vi "PicoScope4000aAWG.vi"(6 "Arbitrary Waveform Settings":T1 {"Index Mode" items=["Single", "Dual", "Quad"]}, 7 "Standard Waveform Settings":T2={"Start Frequency (Hz)"=1000.0, "Stop Frequency (Hz)"=1000.0, "Increment (Hz)"=0.0, "Dwell Time (seconds)"=0.0} {"Start Frequency (Hz)" min=1.0 max=1000000.0}, 8 "error in":errorcluster, 9 "General AWG Settings":T3={"Peak-to-Peak Voltage (microvolts)"=2000000, "Offset Voltage (microvolts)"=0, "Wave Type"=0, "Sweep Type"=0, "Shots"=0, "Sweeps"=0, "Trigger Type"=0, "Trigger Source"=0, "Ext. Threshold (ADC count)"=0, "White Noise/PRBS"=0} {"White Noise/PRBS" items=["Normal", "White Noise", "PRBS"]; "Trigger Source" items=["None", "Scope Trigger", "Aux. In", "Ext. In", "Software Trigger"]; "Trigger Type" items=["Rising", "Falling", "Gate High", "Gate Low"]; "Sweep Type" items=["Up", "Down", "Up-Down", "Down-Up"]; "Wave Type" items=["Sine", "Square", "Triangle", "Ramp Up", "Ramp Down", "Sinc", "Gaussian", "Half Sine", "DC", "Arbitrary"]}, 11 "Handle In":i16) -> (0 "error out":errorcluster, 1 "Arbitrary\nWaveform Graph":i16[](graph), 2 "Trigger Source Out":u32, 3 "Handle Out":i16)   [LabVIEW 2010]
doc: "This VI can be used to control the arbitrary waveform generator. Standard waveforms can be selected or arbitrary waveform can be selected under 'Wave Type'. There are three settings clusters: general settings that apply to both arbitrary and standard waveforms, settings that apply only to standard waveforms and settings that apply only to arbitrary waveforms. It is not necessary to connect all of these clusters if only using arbitrary waveforms or only using standard waveforms are required.\n\nWhen selecting arbitrary waveform, it is necessary to specify a text file containing the wave form. This text file should have a single value on each line in the range -1 to 1. For further information on the settings, see descriptions of ps3000aSetSigGenBuiltIn and ps3000aSetSigGenArbitrary."
uses:
  ps4000A.dll
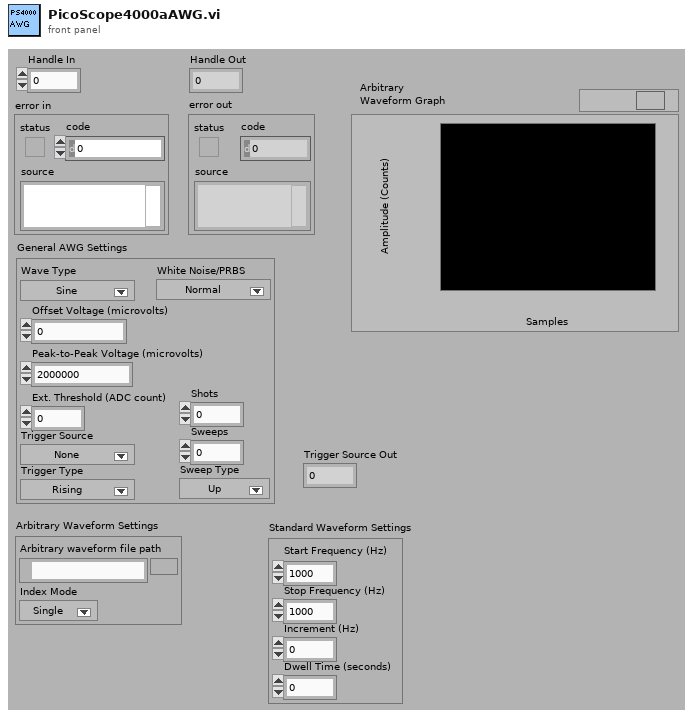
[diagram p1: front panel]
types:
  T1 = cluster{"Arbirary waveform file path":path, "Index Mode":u32}
  T2 = cluster{"Start Frequency (Hz)":dbl, "Stop Frequency (Hz)":dbl, "Increment (Hz)":dbl, "Dwell Time (seconds)":dbl}
  T3 = cluster{"Peak-to-Peak Voltage (microvolts)":u32, "Offset Voltage (microvolts)":i32, "Wave Type":u32, "Sweep Type":u32, "Shots":u32, "Sweeps":u32, "Trigger Type":u32, "Trigger Source":u32, "Ext. Threshold (ADC count)":i16, "White Noise/PRBS":u32}
  T4 = cluster{"status":bool, "code":u32, "source":string}
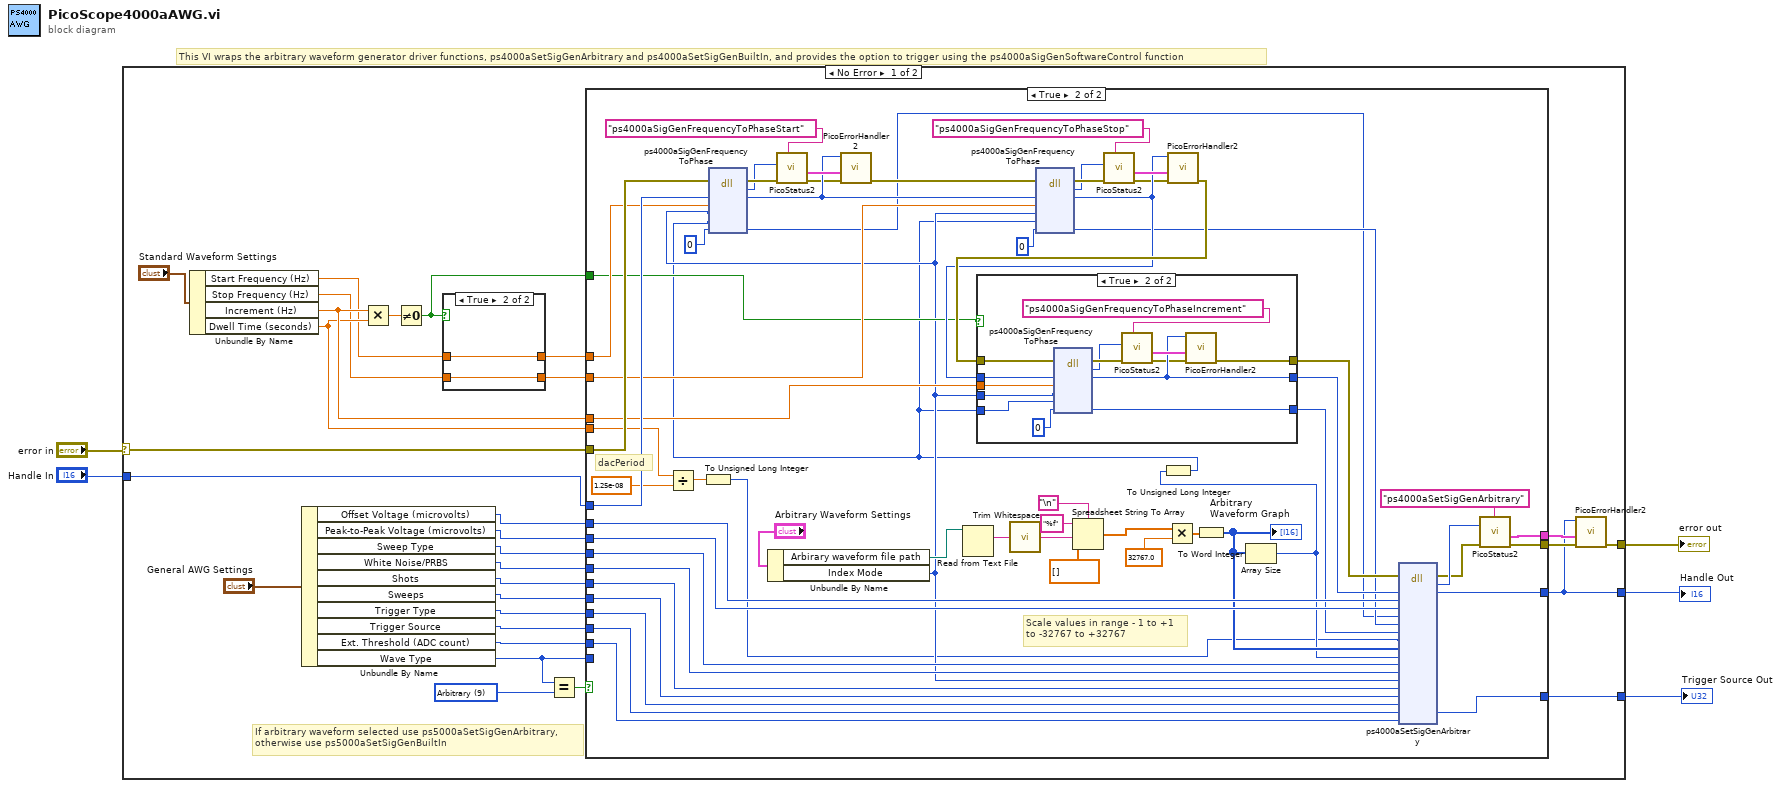
[diagram p0: block diagram]
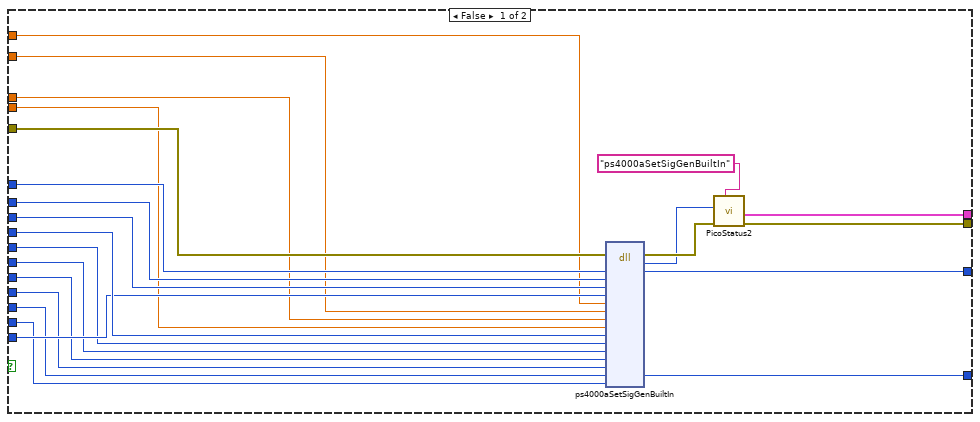
[diagram p3: hidden frame]
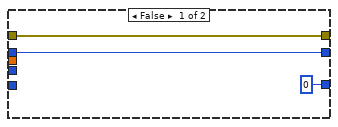
[diagram p4: hidden frame]
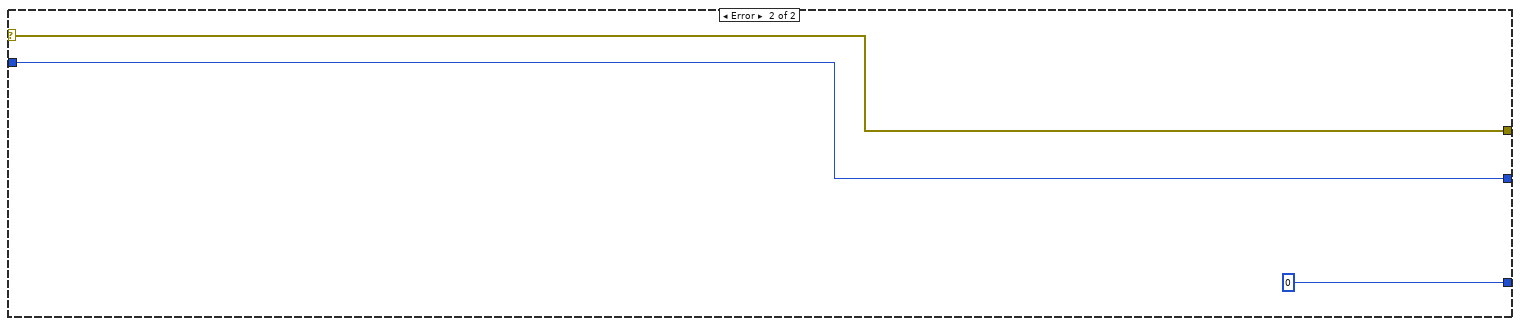
[diagram p5: hidden frame]
diagram:
  # "This VI wraps the arbitrary waveform generator driver functions, ps4000aSetSigGenArbitrary and ps4000aSetSigGenBuiltIn, and provides the option to trigger using the ps4000aSigGenSoftwareControl function"
  n1 = case shown="No Error" "error in" {
    selector: "error in" -> [w21 w141]
    tunnel: [w17 w140] -> w5
    tunnel: "Handle In" -> [w33 w140]
    tunnel: [w32 w141] -> w3
    tunnel: [w19 0] -> w1
    frame No Error {
      w7 = u32 9 items=["Sine", "Square", "Triangle", "Ramp Up", "Ramp Down", "Sinc", "Gaussian", "Half Sine", "DC", "Arbitrary"] ("Wave Type")
      # "If arbitrary waveform selected use ps5000aSetSigGenArbitrary, \notherwise use ps5000aSetSigGenBuiltIn"
      n2 = Unbundle By Name("Standard Waveform Settings") -> ("Start Frequency (Hz)"=w11:dbl, "Stop Frequency (Hz)"=w12:dbl, "Increment (Hz)"=w15:dbl, "Dwell Time (seconds)"=w14:dbl)
      n3 = Unbundle By Name("General AWG Settings") -> ("Offset Voltage (microvolts)"=w30:i32, "Peak-to-Peak Voltage (microvolts)"=w29:u32, "Sweep Type"=w28:u32, "White Noise/PRBS"=w27:u32, "Shots"=w26:u32, "Sweeps"=w25:u32, "Trigger Type"=w24:u32, "Trigger Source"=w23:u32, "Ext. Threshold (ADC count)"=w22:i16, "Wave Type"=w6:u32)
      n4 = Multiply(x=w15, y=w14) -> (x*y=w13:dbl)
      n5 = Not Equal To 0?(x=w13) -> (x != 0?=w8:bool)
      n6 = case shown="True" w8 {
        tunnel: [w35 w37] -> w10
        tunnel: w12 -> [_ w37]
        tunnel: w11 -> [w35 w36]
        tunnel: [w35 w36] -> w9
        frame False {
        }
        frame True {
        }
      }
      n7 = Equal?(x=w6, y=w7) -> (x = y?=w34:bool)
      n8 = case shown="True" w34 {
        tunnel: [w60 w116] -> w17
        tunnel: w33 -> [w59 w79]
        tunnel: [w45 w113] -> w20
        tunnel: w30 -> [w58 w112]
        tunnel: w29 -> [w57 w111]
        tunnel: w28 -> [w56 w110]
        tunnel: w27 -> [w47 w98]
        tunnel: w26 -> [w54 w109]
        tunnel: w25 -> [w53 w108]
        tunnel: w24 -> [w52 w107]
        tunnel: w23 -> [w51 w106]
        tunnel: w22 -> [w50 w103]
        tunnel: w6 -> [w55 _]
        tunnel: [w49 w101] -> w19
        tunnel: w21 -> [w48 w78]
        tunnel: [w44 w95] -> w18
        tunnel: w15 -> [w41 w72]
        tunnel: w14 -> [w40 w63]
        tunnel: w10 -> [w39 w73]
        tunnel: w9 -> [w38 w74]
        tunnel: w8 -> [_ w71]
        frame False {
          n9 = dll-call lib="ps4000A.dll" fn="ps4000aSetSigGenBuiltIn" ("ps3000.dll:_ps3000_open_unit@0")(error in=w48, "handle"=w59, "offsetVoltage"=w58, "pkToPk"=w57, "waveType"=w55, "startFrequency"=w38, "stopFrequency"=w39, "increment"=w41, "dwellTime"=w40, "sweepType"=w56, "operation"=w47, "shots"=w54, "sweeps"=w53, "triggerType"=w52, "triggerSource"=w51, "extInThreshold"=w50) -> (error out=w46:errorcluster, "PICO_STATUS"=w43:u32, "handle"=w60:i16, "triggerSource"=w49:u32)  [unwired: 15 in, 1 out]
          n10 = call "PicoStatus2.vi"("PICO source"="ps4000aSetSigGenBuiltIn" ("source"), "Error in"=w46, "PICO STATUS"=w43) -> ("error out"=w45:errorcluster, "PICO_STATUS out"=w44:T4)  [unwired: 5 in]
        }
        frame True {
          # "dacPeriod"
          # "Scale values in range - 1 to +1 \nto -32767 to +32767"
          n11 = Divide(x=w63, y=1.25e-08) -> (x/y=w65:dbl)
          n12 = To Unsigned Long Integer(number=w65) -> (unsigned 32bit integer=w64:u32)
          n13 = Unbundle By Name("Arbitrary Waveform Settings") -> ("Arbirary waveform file path"=w104:path, "Index Mode"=w70:u32)
          n14 = Read from Text File(file (use dialog)=w104) -> (text=w97:string)  [unwired: 3 in, 3 out]
          n15 = call <vilib>:"Trim Whitespace.vi"("string"=w97) -> ("trimmed string"=w96:string)  [unwired: 1 in]
          n16 = Spreadsheet String To Array(delimiter (Tab)="\n", format string="%f", spreadsheet string=w96, array type (2D Dbl)=dbl[] []) -> (array=w117:dbl[])
          n17 = Multiply(x=w117, y=32767.0 ("deltaPhaseIncrement")) -> (x*y=w99:dbl[])
          n18 = To Word Integer(number=w99) -> (16bit integer=w102:i16[])
          "Arbitrary\nWaveform Graph" <- w102
          n19 = Array Size(array=w102) -> (size(s)=w69:i32)
          n20 = To Unsigned Long Integer(number=w69) -> (unsigned 32bit integer=w68:u32)
          n21 = dll-call lib="ps4000a.dll" fn="ps4000aSigGenFrequencyToPhase" ("ps3000.dll:_ps3000_open_unit@0")(error in=w78, "handle"=w79, "frequency"=w74, "indexMode"=w70, "bufferLength"=w68, "phase"=u32 0) -> (error out=w93:errorcluster, "PICO_STATUS"=w91:u32, "handle"=w81:i16, "phase"=w61:u32)  [unwired: 5 in, 1 out]
          n22 = call "PicoStatus2.vi"("PICO source"="ps4000aSigGenFrequencyToPhaseStart" ("source"), "Error in"=w93, "PICO STATUS"=w91) -> ("error out"=w75:errorcluster, "PICO_STATUS out"=w92:T4)  [unwired: 5 in]
          n23 = call "PicoErrorHandler2.vi"("error in (no error)"=w75, "PICO_STATUS in"=w92, "handle In"=w81) -> ("error out"=w83:errorcluster)  [unwired: 8 in]
          n24 = dll-call lib="ps4000a.dll" fn="ps4000aSigGenFrequencyToPhase" ("ps3000.dll:_ps3000_open_unit@0")(error in=w83, "handle"=w81, "frequency"=w73, "indexMode"=w70, "bufferLength"=w68, "phase"=u32 0) -> (error out=w88:errorcluster, "PICO_STATUS"=w86:u32, "handle"=w80:i16, "phase"=w66:u32)  [unwired: 5 in, 1 out]
          n25 = call "PicoStatus2.vi"("PICO source"="ps4000aSigGenFrequencyToPhaseStop" ("source"), "Error in"=w88, "PICO STATUS"=w86) -> ("error out"=w76:errorcluster, "PICO_STATUS out"=w87:T4)  [unwired: 5 in]
          n26 = call "PicoErrorHandler2.vi"("error in (no error)"=w76, "PICO_STATUS in"=w87, "handle In"=w80) -> ("error out"=w82:errorcluster)  [unwired: 8 in]
          n27 = case shown="True" w71 {
            tunnel: [w124 w134] -> w94
            tunnel: w82 -> [w124 w132]
            tunnel: w80 -> [w123 w131]
            tunnel: [w123 w130] -> w77
            tunnel: w72 -> [_ w128]
            tunnel: w68 -> [_ w127]
            tunnel: w70 -> [_ w126]
            tunnel: [u32 0 ("phase") w125] -> w67
            frame False {
            }
            frame True {
              n28 = dll-call lib="ps4000a.dll" fn="ps4000aSigGenFrequencyToPhase" ("ps3000.dll:_ps3000_open_unit@0")(error in=w132, "handle"=w131, "frequency"=w128, "indexMode"=w126, "bufferLength"=w127, "phase"=u32 0) -> (error out=w138:errorcluster, "PICO_STATUS"=w136:u32, "handle"=w130:i16, "phase"=w125:u32)  [unwired: 5 in, 1 out]
              n29 = call "PicoStatus2.vi"("PICO source"="ps4000aSigGenFrequencyToPhaseIncrement" ("source"), "Error in"=w138, "PICO STATUS"=w136) -> ("error out"=w129:errorcluster, "PICO_STATUS out"=w137:T4)  [unwired: 5 in]
              n30 = call "PicoErrorHandler2.vi"("error in (no error)"=w129, "PICO_STATUS in"=w137, "handle In"=w130) -> ("error out"=w134:errorcluster)  [unwired: 8 in]
            }
          }
          n31 = dll-call lib="ps4000A.dll" fn="ps4000aSetSigGenArbitrary" ("ps3000.dll:_ps3000_open_unit@0")(error in=w94, "handle"=w77, "offsetVoltage"=w112, "pkToPk"=w111, "startDeltaPhase"=w61, "stopDeltaPhase"=w66, "deltaPhaseIncrement"=w67, "dwellCount"=w64, "arbitraryWaveform"=w102, "arbitraryWaveformSize"=w69, "sweepType"=w110, "operation"=w98, "indexMode"=w70, "shots"=w109, "sweeps"=w108, "triggerType"=w107, "triggerSource"=w106, "extInThreshold"=w103) -> (error out=w100:errorcluster, "PICO_STATUS"=w115:u32, "handle"=w116:i16, "triggerSource"=w101:u32)  [unwired: 17 in, 1 out]
          n32 = call "PicoStatus2.vi"("PICO source"="ps4000aSetSigGenArbitrary" ("source"), "Error in"=w100, "PICO STATUS"=w115) -> ("error out"=w113:errorcluster, "PICO_STATUS out"=w95:T4)  [unwired: 5 in]
        }
      }
      n33 = call "PicoErrorHandler2.vi"("error in (no error)"=w20, "PICO_STATUS in"=w18, "handle In"=w17) -> ("error out"=w32:errorcluster)  [unwired: 8 in]
    }
    frame Error {
    }
  }
  "Handle Out" <- w5
  "error out" <- w3
  "Trigger Source Out" <- w1
